vi "lvcsm File Path.vi"() -> (1 "Appended Path":path)   [LabVIEW 2017, in "lvcsm File Support.lvlib"]
uses:
  lvcsm File Support.lvlib
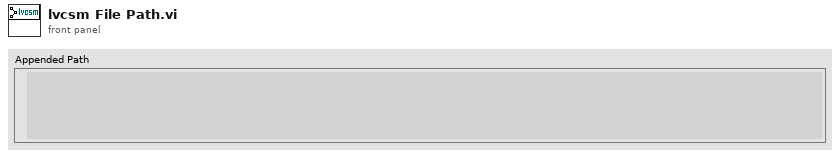
[diagram p1: front panel]
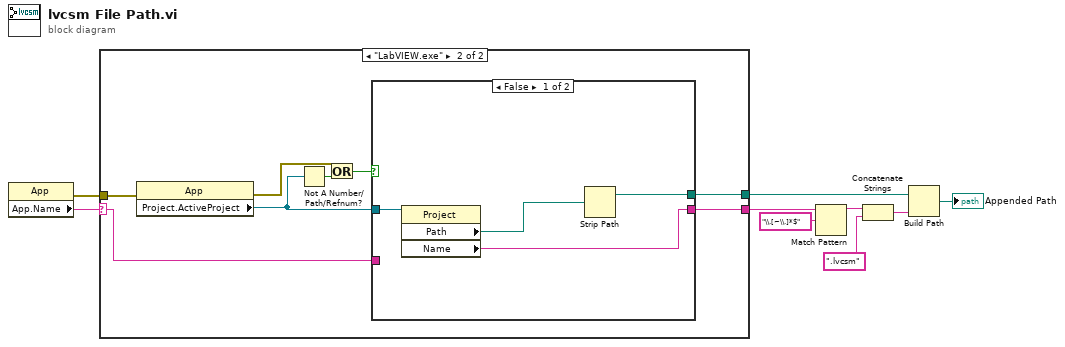
[diagram p0: block diagram]
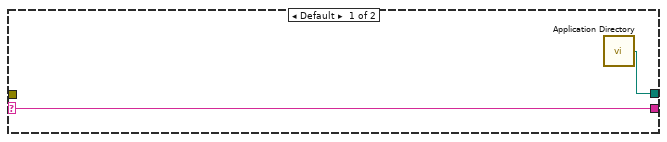
[diagram p2: hidden frame]
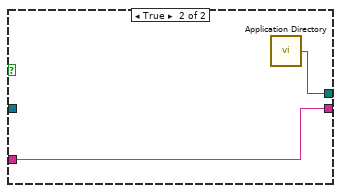
[diagram p3: hidden frame]
diagram:
  n1 = property class="App"() -> (error out=w8:errorcluster, "App.Name"=w9:string)  [unwired: 2 in, 1 out]
  n2 = case shown="\"LabVIEW.exe\"" w9 {
    selector: w9 -> [w11 w13]
    tunnel: w8 -> [_ w17]
    tunnel: [w11 w14] -> w6
    tunnel: [w10 w12] -> w1
    frame Default {
      n3 = call <vilib>:"Application Directory.vi"() -> ("Application Directory"=w10:path)
    }
    frame "LabVIEW.exe" {
      n4 = property class="App"(error in=w17) -> (error out=w19:errorcluster, "Project.ActiveProject"=w16:refnum<vi>)  [unwired: 1 in, 1 out]
      n5 = Not A Number/Path/Refnum?(number/path/refnum=w16) -> (NaN/Path/Refnum?=w18:bool)
      n6 = Or(x=w19, y=w18) -> (x .or. y?=w15:bool)
      n7 = case shown="False" w15 {
        tunnel: w16 -> [w23 _]
        tunnel: [w22 w25] -> w14
        tunnel: w13 -> [_ w25]
        tunnel: [w20 w24] -> w12
        frame False {
          n8 = property class="Project"(reference=w23) -> ("Path"=w21:path, "Name"=w22:string)  [unwired: 1 in, 2 out]
          n9 = Strip Path(path=w21) -> (stripped path=w20:path)  [unwired: 1 out]
        }
        frame True {
          n10 = call <vilib>:"Application Directory.vi"() -> ("Application Directory"=w24:path)
        }
      }
    }
  }
  n11 = Match Pattern(string=w6, regular expression="\\.[~\\.]*$") -> (before substring=w4:string)  [unwired: 1 in, 3 out]
  n12 = Concatenate Strings(w4, ".lvcsm" ("new ending (none)")) -> (w3:string)
  n13 = Build Path(base path=w1, name or relative path=w3) -> (appended path=→"Appended Path":path)
